vi "UI.vi"(8 "error in (no error)":errorcluster, 11 "Node Ptr":T1 format="%.0x") -> (0 "error out":errorcluster)   [LabVIEW 2020, in "Modules.lvlib" / "9253.lvclass"]
uses:
  9253.lvclass
  <vilib>/NI VeriStand/Custom Device API/Custom Device Item Ref.ctl
  RSI Module/SubPanel Command.ctl
  C:/Users/nitest/Desktop/Git 2020/niveristand-scan-engine-module-libraries/Source/RSI Module/RSI Module.lvclass
  9253.lvclass/9253.ctl
  RSI Module/RSI Module.lvclass
  <vilib>/NI VeriStand/Custom Device API/Custom Device API.lvlib
panel:
  in  "Butterworth cutoff frequency":u32(ring) items=["4000 Hz", "2000 Hz", "1000 Hz", "500 Hz", "250 Hz", "125 Hz"]
  in  "Filter response":u32(ring) items=["Comb"=0, "Butterworth"=2]
  in  "Butterworth filter order":u32(ring)=1 items=["Order 2"=1, "Order 4"=3]
  in  "Comb frequency":u32(ring) items=["Data rate", "Data rate / 2", "Data rate / 4", "Data rate / 8", "Data rate / 16"]
  in  "Data rate":u32(ring) items=["50.000 kS/s"=0, "33.333 kS/s"=1, "25.000 kS/s"=2, "20.000 kS/s"=3, "16.667 kS/s"=4, "14.286 kS/s"=5, "12.500 kS/s"=6, "11.111 kS/s"=7, "10.000 kS/s"=8, "8.333 kS/s"=9, "7.143 kS/s"=10, "6.250 kS/s"=11, "5.556 kS/s"=12, "5.000 kS/s"=13, "4.545 kS/s"=14, "4.167 kS/s"=15, "3.571 kS/s"=16, "3.125 kS/s"=17, "2.778 kS/s"=18, "2.500 kS/s"=19, "2.273 kS/s"=20, "2.083 kS/s"=21, "2.000 kS/s"=22, "1.786 kS/s"=23, "1.563 kS/s"=24, "1.389 kS/s"=25, "1.250 kS/s"=26, "1.136 kS/s"=27, "1.042 kS/s"=28, "1.000 kS/s"=29, "892.86 S/s"=30, "781.25 S/s"=31, "694.44 S/s"=32, "625.00 S/s"=33, "568.18 S/s"=34, "520.83 S/s"=35, "500.00 S/s"=36, "446.43 S/s"=37, "400.00 S/s"=38, "390.63 S/s"=39, "347.22 S/s"=40, "312.50 S/s"=41, "284.09 S/s"=42, "260.42 S/s"=43, "250.00 S/s"=44, "223.21 S/s"=45, "200.00 S/s"=46, "195.31 S/s"=47, "142.05 S/s"=48, "125.00 S/s"=49, "100.00 S/s"=50, "97.66 S/s"=51, "60.02 S/s"=52, "50.00 S/s"=54, "10.00 S/s"=56]
  out "_Update Chan Settings":bool
  in  "SubPanel Event":refnum<user-event>
  in  "Header":cluster{"Section Name":string}={"Section Name"="NI 9253 Settings"}
  # "Each 9253 module supports field-side power fault detection and channel overcurrent detection.\nThese features are not supported by this custom device."
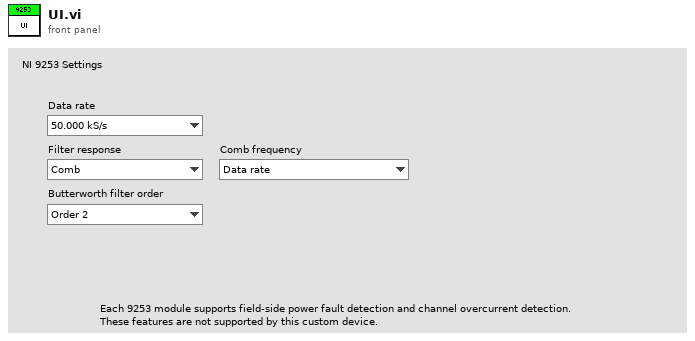
[diagram p1: front panel]
types:
  T1 = typedef "Custom Device API.lvlib/Custom Device Item Ref.ctl" = u64
  T2 = typedef "Modules.lvlib/RSI Module.lvclass/Module Models.ctl" = enum16{"Empty", "NI 9201", "NI 9203", "NI 9205", "NI 9206", "NI 9207", "NI 9208", "NI 9209", "NI 9210", "NI 9211", "NI 9212", "NI 9213", "NI 9214", "NI 9215", "NI 9216", "NI 9217", "NI 9219", "NI 9220", "NI 9221", "NI 9222", "NI 9223", "NI 9224", "NI 9225", "NI 9226", "NI 9227", "NI 9228", "NI 9229", "NI 9233", "NI 9234", "NI 9235", "NI 9236", "NI 9237", "NI 9239", "NI 9242", "NI 9244", "NI 9253", "NI 9263", "NI 9264", "NI 9265", "NI 9266", "NI 9269", "NI 9344", "NI 9350", "NI 9375", "NI 9401", "NI 9402", "NI 9403", "NI 9411", "NI 9421", "NI 9422", "NI 9423", "NI 9425", "NI 9426", "NI 9435", "NI 9436", "NI 9437", "NI 9472", "NI 9474", "NI 9475", "NI 9476", "NI 9477", "NI 9478", "NI 9481", "NI 9482", "NI 9485"}
  T3 = typedef "Modules.lvlib/RSI Module.lvclass/SubPanel Command.ctl" = enum16{"Stop"}
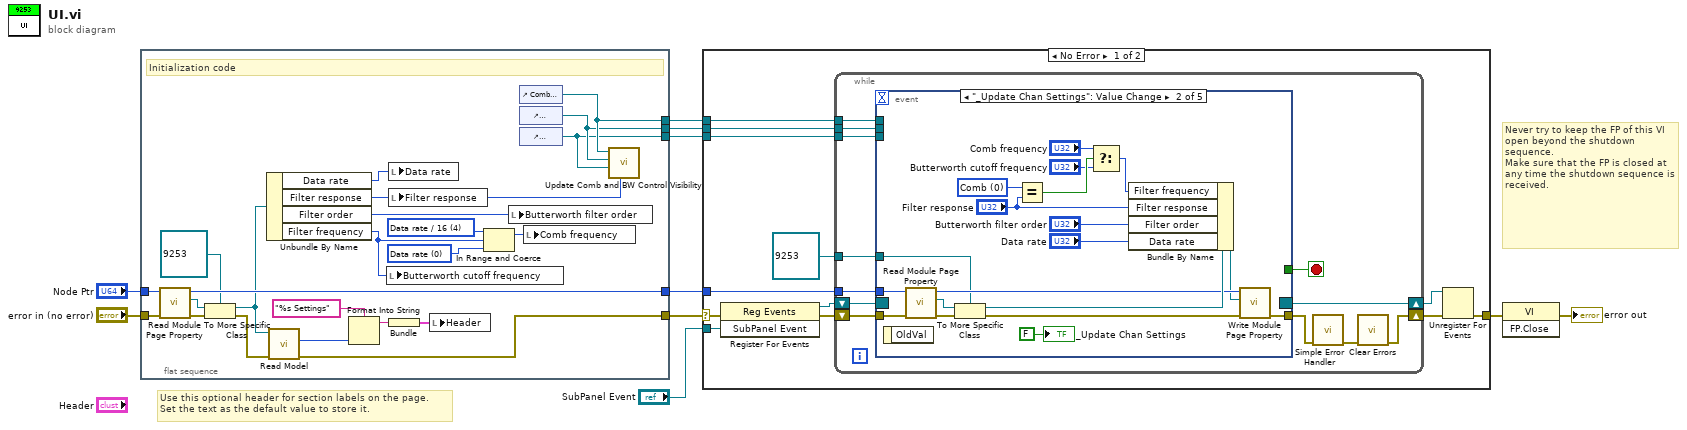
[diagram p0: block diagram]
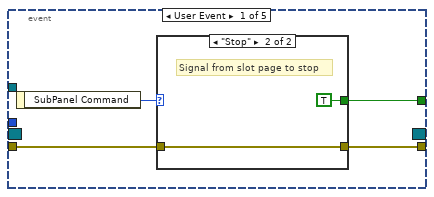
[diagram p2: hidden frame]
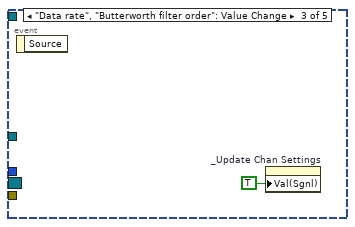
[diagram p4: hidden frame]
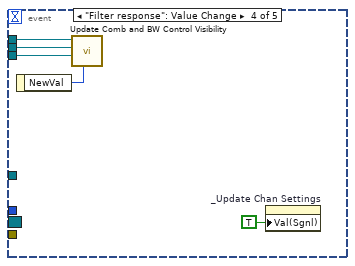
[diagram p5: hidden frame]
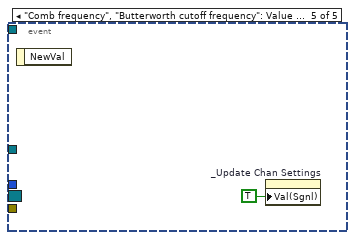
[diagram p6: hidden frame]
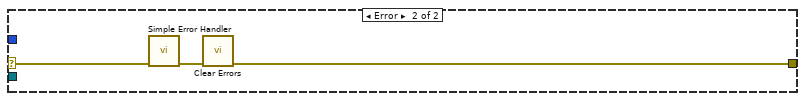
[diagram p7: hidden frame]
diagram:
  # "Never try to keep the FP of this VI open beyond the shutdown sequence.\nMake sure that the FP is closed at any time the shutdown sequence is received."
  # "Use this optional header for section labels on the page. \nSet the text as the default value to store it."
  n1 = flat-sequence {
    tunnel: "error in (no error)" -> [w32]
    tunnel: "Node Ptr" -> [w33]
    tunnel: [w15] -> w4
    tunnel: [w31] -> w7
    tunnel: [w18] -> w3
    tunnel: [w17] -> w2
    tunnel: [w16] -> w1
    frame #0 {
      w12 = u32 0 items=["Data rate", "Data rate / 2", "Data rate / 4", "Data rate / 8", "Data rate / 16"] ("Comb frequency")
      w11 = u32 4 items=["Data rate", "Data rate / 2", "Data rate / 4", "Data rate / 8", "Data rate / 16"] ("Comb frequency")
      # "Initialization code"
      n2 = call "Read Module Page Property.vi"("error in (no error)"=w32, "Node Ptr In"=w33) -> ("error out"=w30:errorcluster, "RSI Module"=w28:refnum<class "RSI Module.lvclass">, "Node Ptr Out"=w31:T1)  [unwired: 7 in]
      n3 = To More Specific Class(target class=refnum<class "9253.lvclass"> refnum ("9205 in"), reference=w28, error in=w30) -> (specific class reference=w27:refnum<class "9253.lvclass">, error out=w26:errorcluster)
      n4 = Unbundle By Name(w27) -> ("Data rate"=w21:u32, "Filter response"=w19:u32, "Filter order"=w20:u32, "Filter frequency"=w14:u32)
      n5 = call "Read Model.vi"("error in (no error)"=w26, "RSI Module in"=w27) -> ("error out"=w15:errorcluster, "Model"=w24:T2)  [unwired: 7 in, 1 out]
      n6 = Format Into String(format string="%s Settings", w24) -> (resulting string=w22:string)  [unwired: 2 in, 1 out]
      n7 = local write "Butterworth cutoff frequency"(w14) -> ()
      n8 = local write "Data rate"(w21) -> ()
      n9 = local write "Filter response"(w19) -> ()
      n10 = Bundle(w22) -> (w25:cluster{string})  [unwired: 1 in]
      n11 = local write "Header"(w25) -> ()
      n12 = In Range and Coerce(upper limit=w11, x=w14, lower limit=w12) -> (coerced(x)=w13:u32)  [unwired: 1 out]
      n13 = local write "Butterworth filter order"(w20) -> ()
      n14 = control-ref of="Comb frequency"() -> (w18:refnum<vi>)
      n15 = control-ref of="Butterworth filter order"() -> (w17:refnum<vi>)
      n16 = control-ref of="Butterworth cutoff frequency"() -> (w16:refnum<vi>)
      n17 = local write "Comb frequency"(w13) -> ()
      n18 = call "Update Comb and BW Control Visibility.vi"("Filter response"=w19, "Butterworth filter order"=w16, "Butterworth cutoff frequency"=w17, "comb frequency"=w18) -> ()  [unwired: 6 in]
    }
  }
  n19 = case shown="No Error" w4 {
    selector: w4 -> [w39 w93]
    tunnel: [w43 w91] -> w10
    tunnel: w7 -> [w40 _]
    tunnel: "SubPanel Event" -> [w38 _]
    tunnel: w3 -> [w37 _]
    tunnel: w2 -> [w36 _]
    tunnel: w1 -> [w35 _]
    frame No Error {
      n20 = register-events(error in=w39, w38) -> (reference out=w41:refnum<event-registration>, error out=w42:errorcluster)  [unwired: 1 in]
      n21 = while {
        tunnel: w40 -> [w53]
        shift-right: [w50] -> w44
        shift-left: w42 -> [w56]
        shift-right: [w57] -> w45
        shift-left: w41 -> [w55]
        tunnel: w37 -> [w49]
        tunnel: w36 -> [w48]
        tunnel: w35 -> [w47]
        tunnel: refnum<class "9253.lvclass"> refnum ("9205 in") -> [w46]
        stop <- w54 stop-if-true
        n22 = event shown="[1] \"_Update Chan Settings\": Value Change" {
          selector: w55 -> [_ _ _ _ _]
          dyn-events: [_ _ _ _ _] -> w57
          timeout: _ -> [_ _ _ _ _]
          tunnel: w56 -> [w60 w76 _ _ _]
          tunnel: [w59 _ _ _ _] -> w54
          tunnel: [w58 w75 _ _ _] -> w52
          tunnel: w53 -> [_ w77 _ _ _]
          tunnel: w49 -> [_ _ _ w87 _]
          tunnel: w48 -> [_ _ _ w86 _]
          tunnel: w47 -> [_ _ _ w85 _]
          tunnel: w46 -> [_ w74 _ _ _]
          event User Event {
            n23 = event-data() -> ("SubPanel Command"=w61:T3)  [unwired: 1 out]
            n24 = case shown="\"Stop\"" w61 {
              tunnel: w60 -> [w62 w63]
              tunnel: [w62 w63] -> w58
              tunnel: [_ TRUE] -> w59
              frame Default {
              }
              frame "Stop" {
                # "Signal from slot page to stop"
              }
            }
          }
          event "_Update Chan Settings": Value Change {
            w72 = u32 0 items=["Comb"=0, "Butterworth"=2] ("Filter response")
            n25 = event-data() -> ()  [unwired: 2 out]
            n26 = call "Read Module Page Property.vi"("error in (no error)"=w76, "Node Ptr In"=w77) -> ("error out"=w82:errorcluster, "RSI Module"=w83:refnum<class "RSI Module.lvclass">, "Node Ptr Out"=w79:T1)  [unwired: 7 in]
            n27 = To More Specific Class(target class=w74, reference=w83, error in=w82) -> (specific class reference=w81:refnum<class "9253.lvclass">, error out=w80:errorcluster)
            n28 = Equal?(x=w72, y="Filter response") -> (x = y?=w70:bool)
            n29 = Select(t="Comb frequency", s=w70, f="Butterworth cutoff frequency") -> (s? t:f=w65:u32)
            n30 = Bundle By Name(cluster=w81, "Filter frequency"=w65, "Filter response"="Filter response", "Filter order"="Butterworth filter order", "Data rate"="Data rate") -> (w78:refnum<class "9253.lvclass">)
            n31 = call "Write Module Page Property.vi"("error in (no error)"=w80, "RSI Module"=w78, "Node Ptr In"=w79) -> ("error out"=w75:errorcluster)  [unwired: 6 in, 2 out]
            "_Update Chan Settings" <- FALSE ("_Update Values")
          }
          event "Data rate", "Butterworth filter order": Value Change {
            n32 = event-data() -> ()  [unwired: 2 out]
            n33 = property on="_Update Chan Settings" class="Bool (strict)"("Val(Sgnl)"=TRUE ("Value (Signaling)")) -> ()  [unwired: 2 in, 2 out]
          }
          event "Filter response": Value Change {
            n34 = event-data() -> ("NewVal"=w88:u32)  [unwired: 1 out]
            n35 = call "Update Comb and BW Control Visibility.vi"("Filter response"=w88, "Butterworth filter order"=w85, "Butterworth cutoff frequency"=w86, "comb frequency"=w87) -> ()  [unwired: 6 in]
            n36 = property on="_Update Chan Settings" class="Bool (strict)"("Val(Sgnl)"=TRUE ("Value (Signaling)")) -> ()  [unwired: 2 in, 2 out]
          }
          event "Comb frequency", "Butterworth cutoff frequency": Value Change {
            n37 = event-data() -> ()  [unwired: 2 out]
            n38 = property on="_Update Chan Settings" class="Bool (strict)"("Val(Sgnl)"=TRUE ("Value (Signaling)")) -> ()  [unwired: 2 in, 2 out]
          }
        }
        n39 = call <vilib>:"Simple Error Handler.vi"("error in (no error)"=w52) -> ("error out"=w51:errorcluster)  [unwired: 1 in, 7 out]
        n40 = call <vilib>:"Clear Errors.vi"("error in (no error)"=w51) -> ("error out"=w50:errorcluster)  [unwired: 1 in, 5 out]
      }
      n41 = Unregister For Events(event registration refnum=w45, error in=w44) -> (error out=w43:errorcluster)
    }
    frame Error {
      n42 = call <vilib>:"Simple Error Handler.vi"("error in (no error)"=w93) -> ("error out"=w92:errorcluster)  [unwired: 1 in, 7 out]
      n43 = call <vilib>:"Clear Errors.vi"("error in (no error)"=w92) -> ("error out"=w91:errorcluster)  [unwired: 1 in, 5 out]
    }
  }
  n44 = invoke class="VI" method="FP.Close"(error in=w10) -> (error out=→"error out":errorcluster)  [unwired: 2 in, 2 out]
